vi "Run.vi"(8 "error in (no error)":errorcluster, 10 "UI Refs":T1, 11 "Pressure Gain":refnum<class "Pressure Gain.lvclass">) -> (0 "error out":errorcluster, 3 "Pressure Gain out":refnum<class "Pressure Gain.lvclass">)   [LabVIEW 2025, in "Flow Grind.lvlib" / "Pressure Gain.lvclass"]
uses:
  Pressure Gain.lvclass
  Pressure Gain.lvclass/Pressure Gain.ctl
  Users/Public/Documents/Sandia National Labs/TSS Plugin/Tests/XY Plotter.lvlibp/XY  Plotter/XY Plotter.lvclass
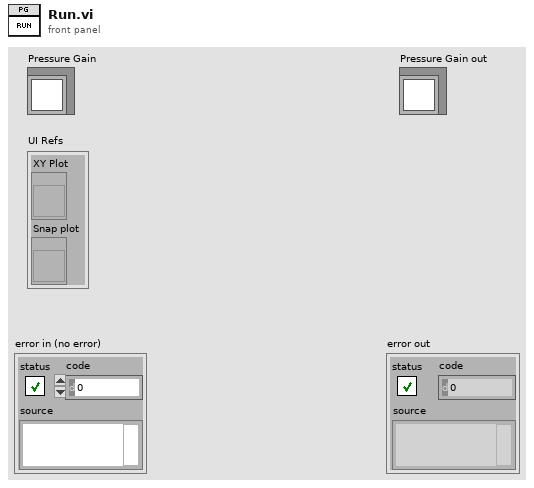
[diagram p1: front panel]
types:
  T1 = cluster{"XY Plot":refnum<vi>, "Snap plot":refnum<vi>}
  T2 = cluster{"Name":string, "Color":u32, "Style":u8, "Point Style":u8, "Name Visible":bool, "Allow Drag":bool, "Annotation Mode":u32, "Plot":i32, "Index":i32, "Position":cluster{"X":dbl, "Y":dbl}, "X Scale":u32, "Y Scale":u32, "Show Arrow":bool, "Lock Name":bool, "Plot Area":i32, "Label Offset":cluster{"X":dbl, "Y":dbl}}
  T3 = typedef "LVAnnotationListTypeDef.ctl" = cluster{"Name":string, "Color":u32, "Style":u8, "Point Style":u8, "Name Visible":bool, "Allow Drag":bool, "Annotation Mode":u32, "Plot":i32, "Index":i32, "Position":cluster{"X":dbl, "Y":dbl}, "X Scale":u32, "Y Scale":u32, "Show Arrow":bool, "Lock Name":bool, "Plot Area":i32, "Label Offset":cluster{"X":dbl, "Y":dbl}}[]
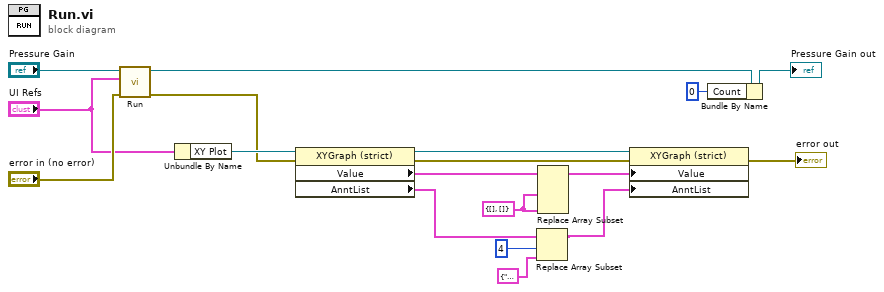
[diagram p0: block diagram]
diagram:
  w5 = cluster{"Wavenumber":dbl[], "Data":dbl[]} {"Wavenumber"=[], "Data"=[]} ("Spectrum")
  n1 = call-parent "Run.vi"("error in (no error)"="error in (no error)", "UI Refs"="UI Refs", "XY Plotter"="Pressure Gain") -> ("error out"=w9:errorcluster, "XY Plotter out"=w17:refnum<class "Pressure Gain.lvclass">)  [unwired: 7 in]
  n2 = Unbundle By Name("UI Refs") -> ("XY Plot"=w11:refnum<vi>)
  n3 = property class="XYGraph (strict)"(reference=w11) -> (reference out=w12:refnum<vi>, "Value"=w13:cluster{"Wavenumber":dbl[], "Data":dbl[]}[], "AnntList"=w4:T3)  [unwired: 1 in, 1 out]
  n4 = Replace Array Subset(array=w4, new element=T2 {"Name"="", "Color"=0, "Style"=0, "Point Style"=0, "Name Visible"=FALSE, "Allow Drag"=FALSE, "Annotation Mode"=0, "Plot"=0, "Index"=0, "Position"={"X"=0.0, "Y"=0.0}, "X Scale"=0, "Y Scale"=0, "Show Arrow"=FALSE, "Lock Name"=FALSE, "Plot Area"=0, "Label Offset"={"X"=0.0, "Y"=0.0}} ("new element/subarray"), index=4) -> (w3:T3)
  n5 = Replace Array Subset(array=w13, new element #1=w5, new element #2=w5) -> (w14:cluster{"Wavenumber":dbl[], "Data":dbl[]}[])  [unwired: 2 in]
  n6 = property class="XYGraph (strict)"(reference=w12, error in=w9, "Value"=w14, "AnntList"=w3) -> (error out=→"error out":errorcluster)  [unwired: 1 out]
  n7 = Bundle By Name(cluster=w17, "Count"=0) -> (→"Pressure Gain out":refnum<class "Pressure Gain.lvclass">)
